vi "onTestExecution.vi"(6 "timeout (2000 ms)":i32=2000, 7 "Name":string, 8 "error in (no error)":errorcluster, 11 "Test Runner.Collection in":refnum<class "Test Runner.Collection.lvclass">) -> (0 "error out":errorcluster, 3 "Test Runner.Collection out":refnum<class "Test Runner.Collection.lvclass">)   [LabVIEW 2020, in "Caraya.lvlib" / "Test Runner.Collection.lvclass"]
uses:
  Test Runner.Collection.lvclass
  Test Runner.Collection.lvclass/Test Runner.Collection.ctl
  Test Runner/Test Runner.lvclass
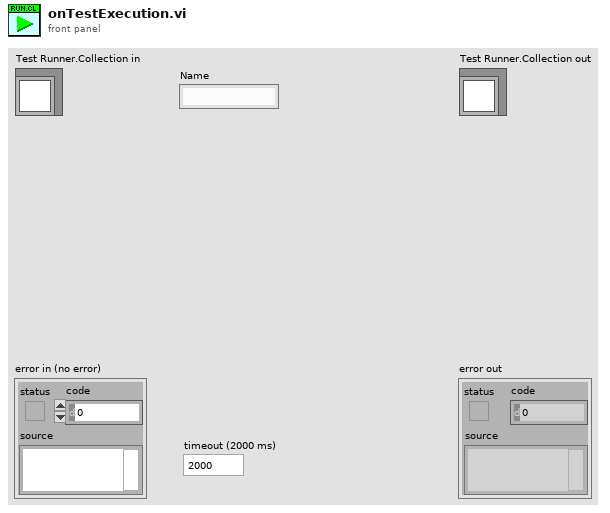
[diagram p1: front panel]
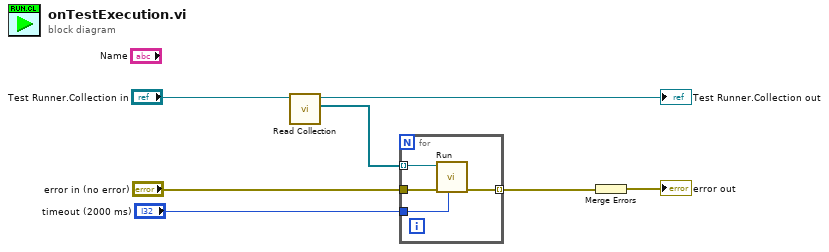
[diagram p0: block diagram]
diagram:
  n1 = call "Read Collection.vi"("Test Runner.Collection in"="Test Runner.Collection in") -> ("Test Runners"=w6:refnum<class "Test Runner.lvclass">[], "Test Runner.Collection out"=→"Test Runner.Collection out":refnum<class "Test Runner.Collection.lvclass">)  [unwired: 9 in]
  n2 = for {
    tunnel: w6 -> [w11] mode=indexing
    tunnel: "error in (no error)" -> [w10]
    tunnel: [w9] -> w7 mode=indexing
    tunnel: "timeout (2000 ms)" -> [w8]
    n3 = call "Run.vi"("timeout"=w8, "error in (no error)"=w10, "Test Runner in"=w11) -> ("error out"=w9:errorcluster)  [unwired: 6 in, 2 out]
  }
  n4 = Merge Errors(w7) -> (→"error out":errorcluster)
